vi "Zad3.vi"() -> ()   [LabVIEW 2025]
panel:
  out "max X":i32
  out "max Z":i32
  out "max Y":i32
  out "AccelerationX":i32
  out "AccelerationZ":i32
  out "AccelerationY":i32
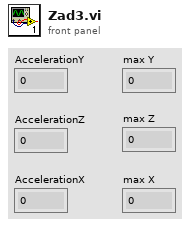
[diagram p1: front panel]
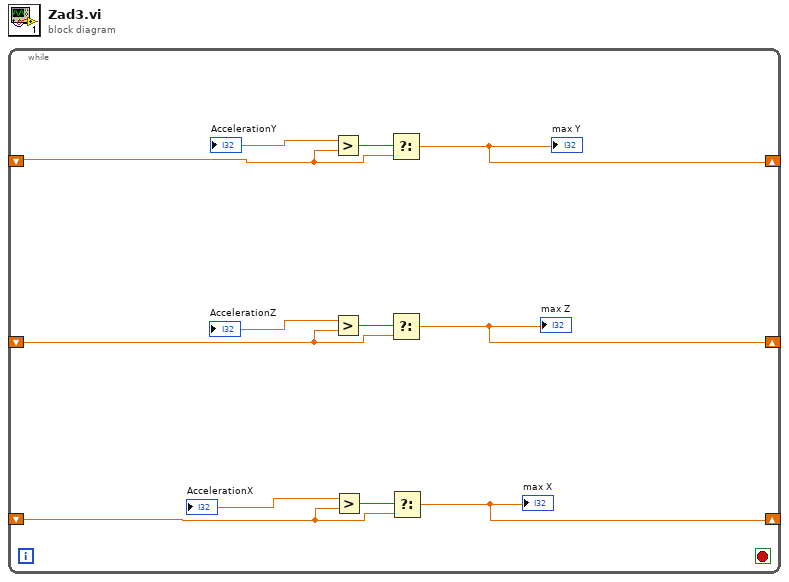
[diagram p0: block diagram]
diagram:
  n1 = while {
    shift-right: [w11] -> _
    shift-left: _ -> [w9]
    shift-right: [w6] -> _
    shift-left: _ -> [w5]
    shift-right: [w2] -> _
    shift-left: _ -> [w1]
    stop <- _ stop-if-true
    n2 = Greater?(y=w1) -> (x=→"AccelerationY":dbl, 0:w4:bool)
    n3 = Greater?(y=w5) -> (x=→"AccelerationZ":dbl, 0:w8:bool)
    n4 = Greater?(y=w9) -> (x=→"AccelerationX":dbl, 0:w12:bool)
    n5 = Select(s=w4, f=w1) -> (s? t:f=w2:dbl)  [unwired: 1 in]
    "max Y" <- w2
    n6 = Select(s=w8, f=w5) -> (s? t:f=w6:dbl)  [unwired: 1 in]
    "max Z" <- w6
    n7 = Select(s=w12, f=w9) -> (s? t:f=w11:dbl)  [unwired: 1 in]
    "max X" <- w11
  }
